vi "Take Snapshot.vi"(8 "error in (no error)":errorcluster, 9 "Timeout (ms) (Default: 10000)":i32=10000, 11 "Camera in":refnum<class "Camera.lvclass">) -> (0 "error out":errorcluster, 2 "New Buffer":refnum<class "Buffer.lvclass">, 3 "Camera":refnum<class "Camera.lvclass">)   [LabVIEW 2020, in "Camera.lvclass"]
doc: "Take a snapshot from the camera. If the camera is setup to require a trigger then this operation will wait for the specified timeout for that trigger to be received and return an <b>Error 56</b> if a timeout occurs.\n\nThe snapshot is returned as a new buffer which can be read and should then be destroyed to free up the underying resources."
uses:
  Camera.lvclass
  Buffer/Buffer.lvclass
  Camera.lvclass/Camera.ctl
  Buffer/Buffer.lvclass/Buffer.ctl
  bin/gindustrialcam_32-1.dll
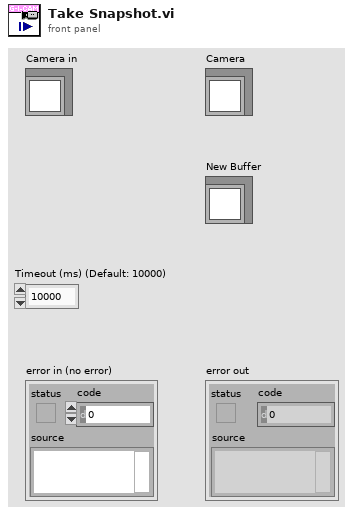
[diagram p1: front panel]
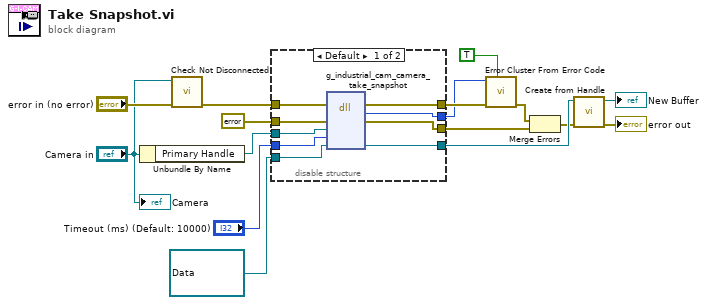
[diagram p0: block diagram]
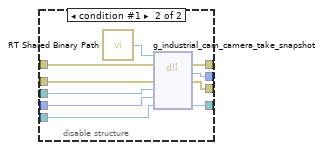
[diagram p2: hidden frame]
diagram:
  n1 = Unbundle By Name("Camera in") -> ("Primary Handle"=w9:refnum<data-value>)
  n2 = call "Check Not Disconnected.vi"("error in (no error)"="error in (no error)", "Camera in"="Camera in") -> ("error out"=w2:errorcluster)  [unwired: 9 in]
  n3 = disable-structure shown="Default" {
    disable-tunnel: [w25 w35] -> w15
    disable-tunnel: [w24 w34] -> w14
    disable-tunnel: [w23 w33] -> w12
    disable-tunnel: errorcluster {"status"=FALSE, "code"=0, "source"=""} ("error constant") -> [w22 w32]
    disable-tunnel: w9 -> [w21 w31]
    disable-tunnel: "Timeout (ms) (Default: 10000)" -> [w20 w30]
    disable-tunnel: refnum<data-value> refnum ("Handle") -> [w19 w29]
    disable-tunnel: [w18 w28] -> w6
    disable-tunnel: w2 -> [w17 w27]
    frame condition #0 (active) {
      n4 = dll-call lib="C:/serenial/lib/g-industrial-camera/LabVIEW/g_industrial_cam/bin/gindustrialcam_*-1.*" fn="g_industrial_cam_camera_take_snapshot"(error in=w17, "err"=w22, "cam_edvr"=w21, "timeout"=w20, "buffer_edvr"=w19) -> (error out=w25:errorcluster, "Mg_Error"=w24:i32, "err"=w23:errorcluster, "buffer_edvr"=w18:refnum<data-value>)  [unwired: 4 in, 1 out]
    }
    frame condition #1 {
      n5 = call "RT Shared Binary Path.vi"() -> ("Path"=w26:path)
      n6 = dll-call lib="C:/serenial/lib/g-industrial-camera/LabVIEW/g_industrial_cam/bin/gindustrialcam_*-1.*" fn="g_industrial_cam_camera_take_snapshot"(path in=w26, error in=w27, "err"=w32, "cam_edvr"=w31, "timeout"=w30, "buffer_edvr"=w29) -> (error out=w35:errorcluster, "Mg_Error"=w34:i32, "err"=w33:errorcluster, "buffer_edvr"=w28:refnum<data-value>)  [unwired: 3 in, 1 out]
    }
  }
  n7 = call <vilib>:"Error Cluster From Error Code.vi"("show call chain? (False)"=TRUE, "error in (no error)"=w15, "error code (0)"=w14) -> ("error out"=w13:errorcluster)  [unwired: 6 in]
  n8 = Merge Errors(w13, w12) -> (w5:errorcluster)
  n9 = call "Create from Handle.vi"("error in (no error)"=w5, "Handle"=w6) -> ("error out"=→"error out":errorcluster, "Buffer out"=→"New Buffer":refnum<class "Buffer.lvclass">)  [unwired: 8 in]
  "Camera" <- "Camera in"
